vi "FuncVI_Sub - Probe - Set Window Position - Global.vi"(8 "error in":errorcluster, 9 "Window Position":cluster{"x":i16, "y":i16}, 11 "VI Refnum":refnum<vi>) -> (0 "error out":errorcluster, 3 "dup VI Refnum":refnum<vi>)   [LabVIEW 2021]
doc: "::: CalcExpress Toolkit :::\nCopyright (c) 2000-2026 Konstantin Shifershteyn. All rights reserved."
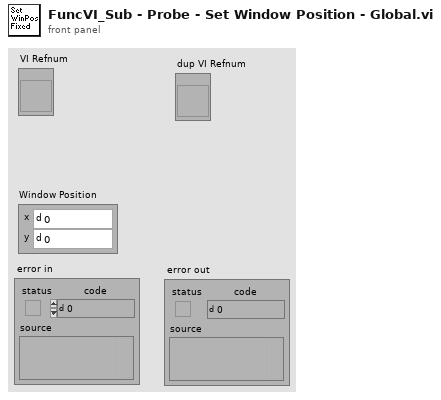
[diagram p1: front panel]
types:
  T1 = typedef "LVAllMonitorsDisplayTypeDef.ctl" = cluster{"Bounds":cluster{"Left":i16, "Top":i16, "Right":i16, "Bottom":i16}, "Depth":i16}[]
  T2 = typedef "LVRectTypeDef.ctl" = cluster{"Left":i16, "Top":i16, "Right":i16, "Bottom":i16}
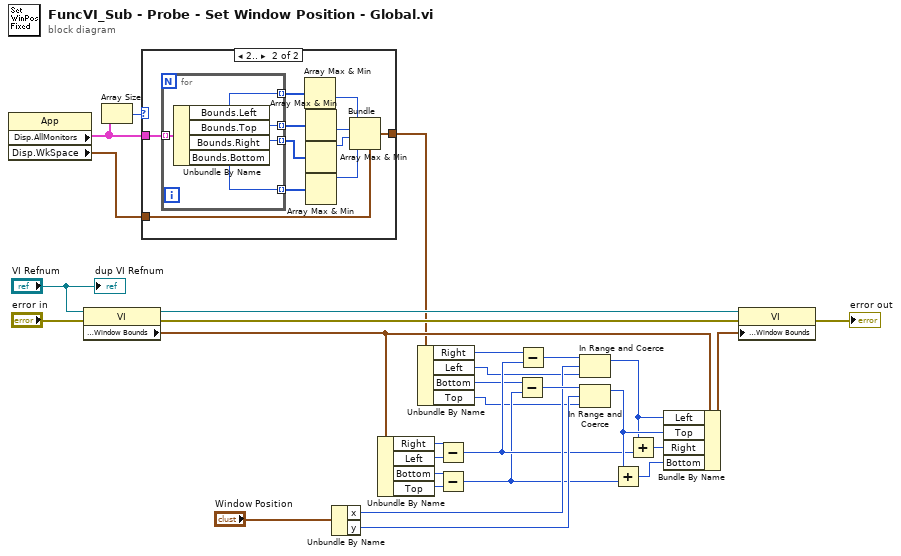
[diagram p0: block diagram]
diagram:
  n1 = property class="App"() -> ("Disp.AllMonitors"=w27:T1, "Disp.WkSpace"=w28:T2)  [unwired: 2 in, 2 out]
  n2 = property class="VI"(reference="VI Refnum", error in="error in") -> (reference out=w25:refnum<vi>, error out=w24:errorcluster, "Front Panel Window:Window Bounds"=w6:T2)
  n3 = Array Size(array=w27) -> (size(s)=w26:i32)
  n4 = case shown="2.." w26 {
    tunnel: w28 -> [w31 w42]
    tunnel: w27 -> [_ w33]
    tunnel: [w31 w32] -> w1
    frame ..1 {
    }
    frame 2.. {
      n5 = for {
        tunnel: w33 -> [w43] mode=indexing
        tunnel: [w47] -> w41 mode=indexing
        tunnel: [w46] -> w40 mode=indexing
        tunnel: [w44] -> w39 mode=indexing
        tunnel: [w45] -> w38 mode=indexing
        n6 = Unbundle By Name(w43) -> ("Bounds.Left"=w47:i16, "Bounds.Top"=w46:i16, "Bounds.Right"=w44:i16, "Bounds.Bottom"=w45:i16)
      }
      n7 = Array Max & Min(array=w41) -> (min value=w37:i16)  [unwired: 3 out]
      n8 = Array Max & Min(array=w40) -> (min value=w36:i16)  [unwired: 3 out]
      n9 = Array Max & Min(array=w39) -> (max value=w35:i16)  [unwired: 3 out]
      n10 = Array Max & Min(array=w38) -> (max value=w34:i16)  [unwired: 3 out]
      n11 = Bundle(cluster=w42, "Left"=w37, "Top"=w36, "Right"=w35, "Bottom"=w34) -> (w32:T2)
    }
  }
  n12 = Unbundle By Name("Window Position") -> ("x"=w15:i16, "y"=w14:i16)
  n13 = Unbundle By Name(w6) -> ("Right"=w10:i16, "Left"=w11:i16, "Bottom"=w12:i16, "Top"=w13:i16)
  n14 = Unbundle By Name(w1) -> ("Right"=w5:i16, "Left"=w4:i16, "Bottom"=w3:i16, "Top"=w2:i16)
  n15 = Subtract(x=w10, y=w11) -> (x-y=w9:i16)
  n16 = Subtract(x=w12, y=w13) -> (x-y=w8:i16)
  n17 = Subtract(x=w3, y=w8) -> (x-y=w17:i16)
  n18 = Subtract(x=w5, y=w9) -> (x-y=w18:i16)
  n19 = In Range and Coerce(upper limit=w18, x=w15, lower limit=w4) -> (coerced(x)=w19:i16)  [unwired: 1 out]
  n20 = In Range and Coerce(upper limit=w17, x=w14, lower limit=w2) -> (coerced(x)=w20:i16)  [unwired: 1 out]
  n21 = Add(x=w20, y=w8) -> (x+y=w22:i16)
  n22 = Add(x=w19, y=w9) -> (x+y=w21:i16)
  n23 = Bundle By Name(cluster=w6, "Left"=w19, "Top"=w20, "Right"=w21, "Bottom"=w22) -> (w7:T2)
  n24 = property class="VI"(reference=w25, error in=w24, "Front Panel Window:Window Bounds"=w7) -> (error out=→"error out":errorcluster)  [unwired: 1 out]
  "dup VI Refnum" <- "VI Refnum"
